vi "InitCSMs.vi"(7 "Enable Conditional Building lvlibp?":bool=TRUE, 8 "error in":errorcluster) -> (0 "error out":errorcluster, 2 "CSMs":string[](array[string]))   [LabVIEW 2017, in "CSM-Testcase.lvlib"]
uses:
  CSM-Testcase.lvlib
  <vilib>/AppBuilder/AB_API_Simple/Build (path).vi
  Chain1.vi
  Chain2.vi
  Chain3.vi
  src/user.lib/_NEVSTOP/Communicable State Machine(CSM)/Communicable State Machine.lvlib
  <vilib>/AppBuilder/AB_API_Simple/NI_App_Builder_API.lvlib
panel:
  out "Waited (ms)":u32
  out "CSMs Left":string[](array[string])
  out "Generated files":path[](array[path])
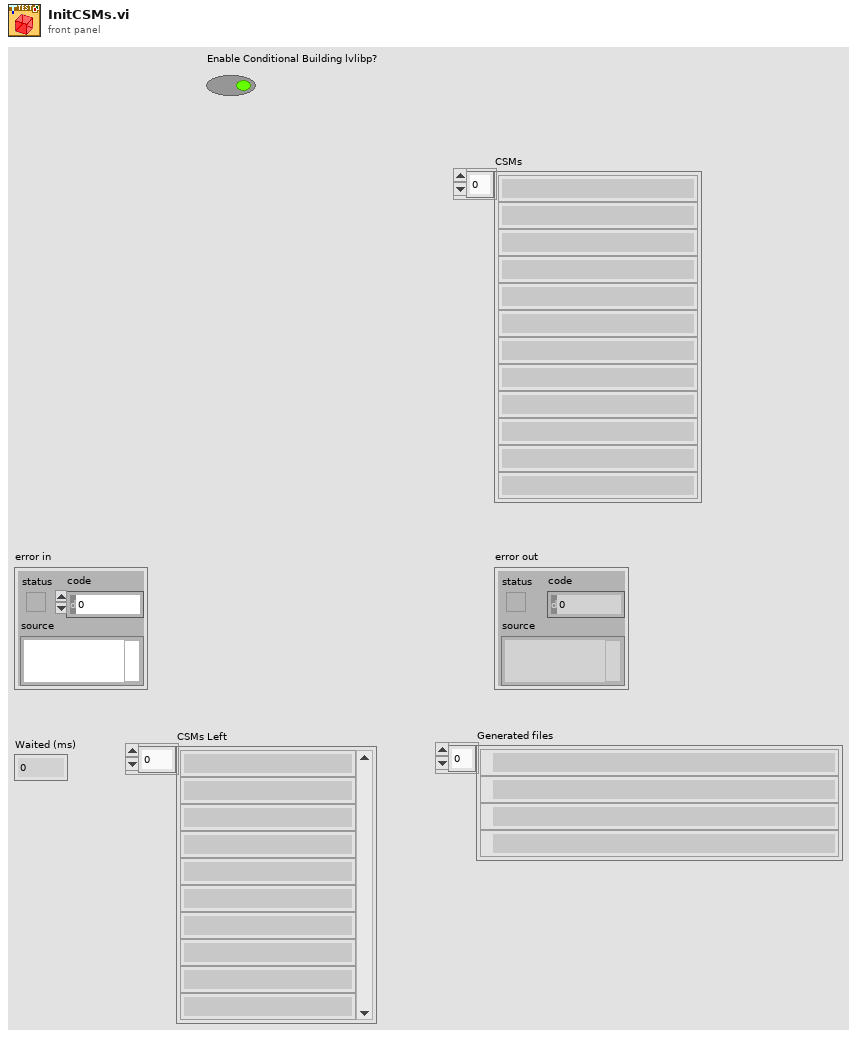
[diagram p1: front panel]
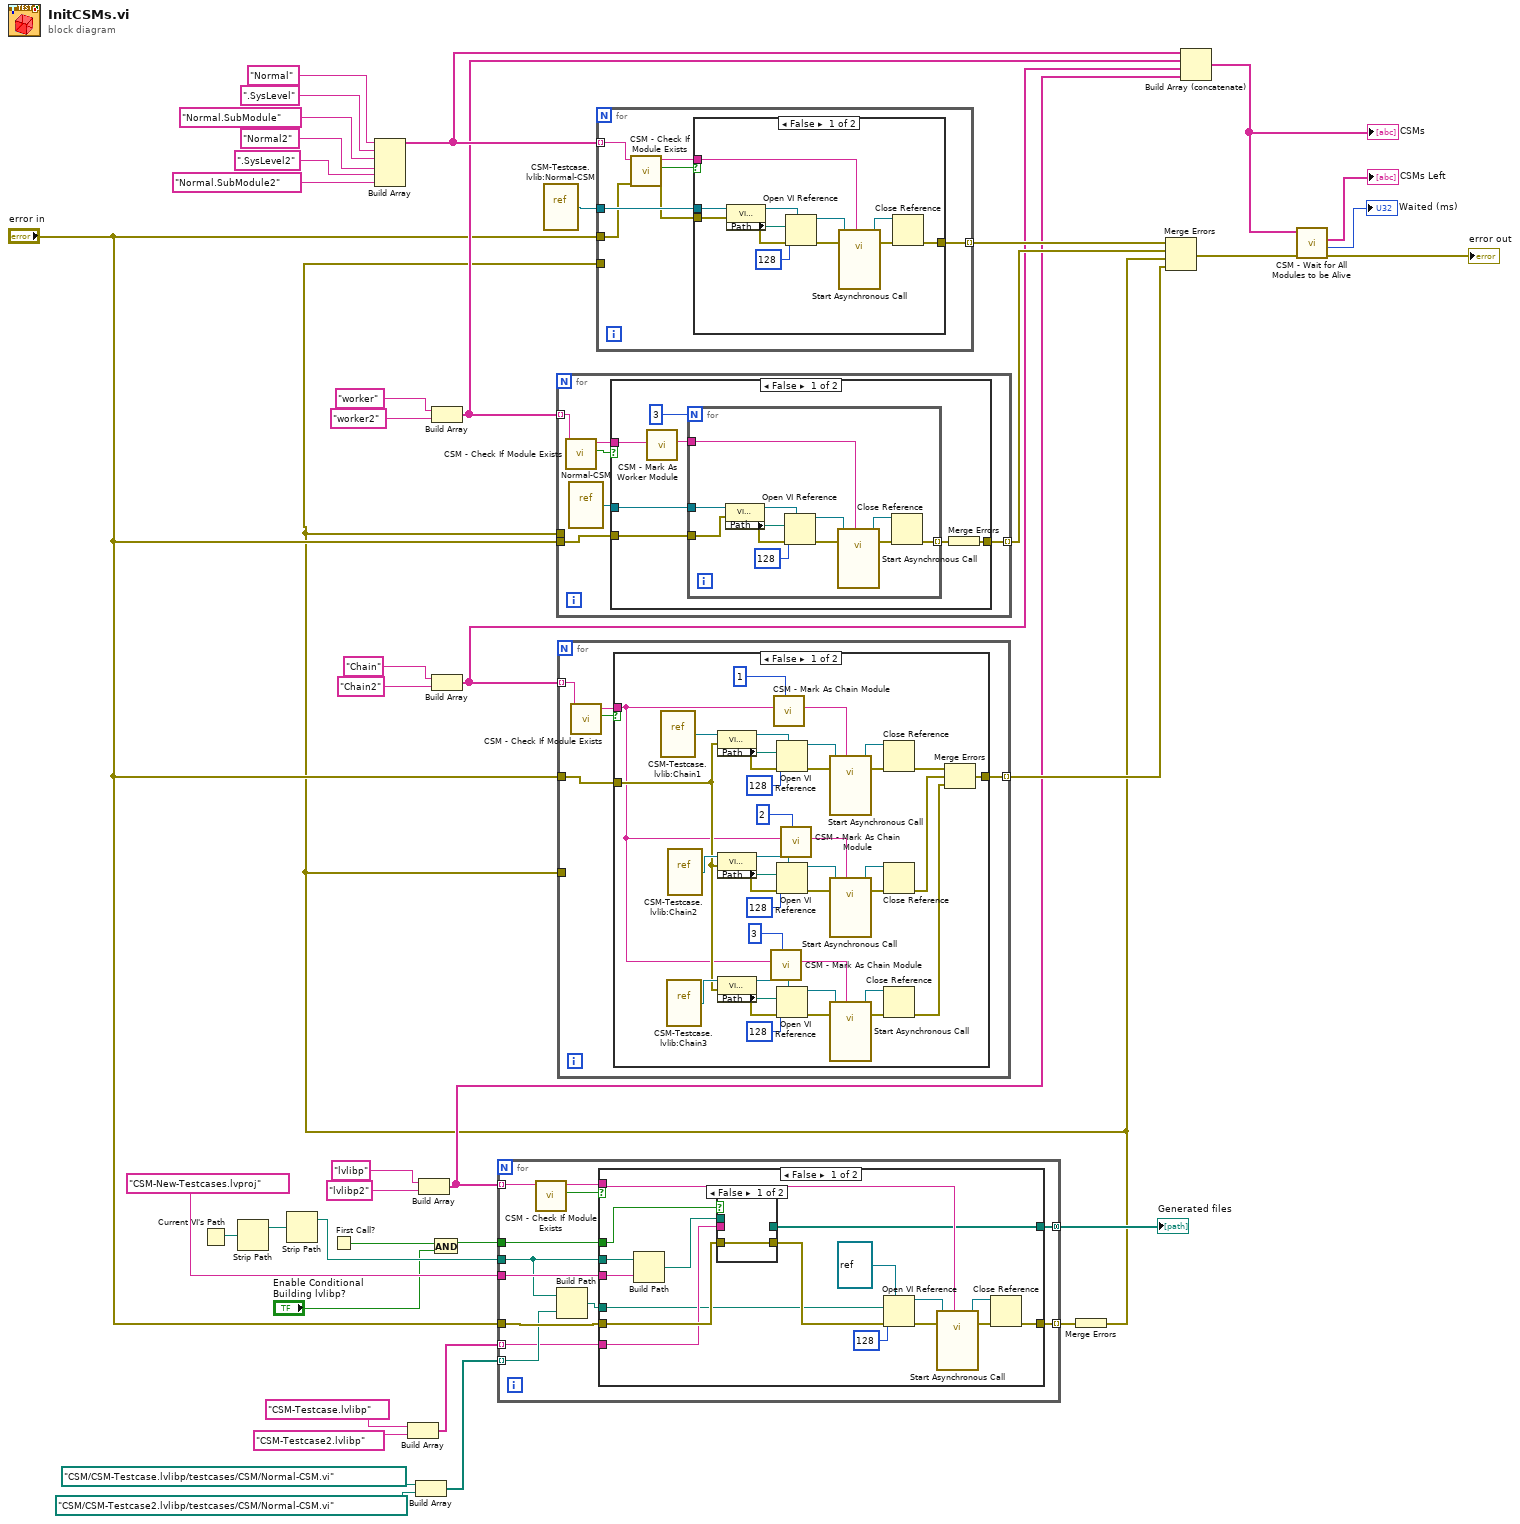
[diagram p0: block diagram]
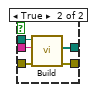
[diagram p2: hidden frame]
diagram:
  n1 = Current VI's Path() -> (path=w38:path)
  n2 = Strip Path(path=w38) -> (stripped path=w39:path)  [unwired: 1 out]
  n3 = Strip Path(path=w39) -> (stripped path=w40:path)  [unwired: 1 out]
  n4 = First Call?() -> (First Call?: T/F=w4:bool)
  n5 = Build Array("Normal" ("Name (\"\" to Use UUID)"), ".SysLevel" ("Name (\"\" to Use UUID)"), "Normal.SubModule" ("Name (\"\" to Use UUID)"), "Normal2" ("Name (\"\" to Use UUID)"), ".SysLevel2" ("Name (\"\" to Use UUID)"), "Normal.SubModule2" ("Name (\"\" to Use UUID)")) -> (w34:string[])
  n6 = Build Array("CSM-Testcase.lvlibp" ("Name of build specification (if empty: build all)"), "CSM-Testcase2.lvlibp" ("Name of build specification (if empty: build all)")) -> (w12:string[])
  n7 = Build Array(path "CSM/CSM-Testcase.lvlibp/testcases/CSM/Normal-CSM.vi" ("vi path"), path "CSM/CSM-Testcase2.lvlibp/testcases/CSM/Normal-CSM.vi" ("vi path")) -> (w15:path[])
  n8 = Build Array("lvlibp" ("Name (\"\" to Use UUID)"), "lvlibp2" ("Name (\"\" to Use UUID)")) -> (w18:string[])
  n9 = And(x=w4, y="Enable Conditional Building lvlibp?") -> (x .and. y?=w3:bool)
  n10 = Build Array("worker" ("Name (\"\" to Use UUID)"), "worker2" ("Name (\"\" to Use UUID)")) -> (w24:string[])
  n11 = Build Array("Chain" ("Name (\"\" to Use UUID)"), "Chain2" ("Name (\"\" to Use UUID)")) -> (w21:string[])
  n12 = for {
    tunnel: "CSM-New-Testcases.lvproj" ("name or relative path") -> [w52]
    tunnel: w40 -> [w47]
    tunnel: w18 -> [w49] mode=indexing
    tunnel: w15 -> [w48] mode=indexing
    tunnel: w12 -> [w45] mode=indexing
    tunnel: [w44] -> w11 mode=concatenating
    tunnel: w3 -> [w43]
    tunnel: "error in" -> [w53]
    tunnel: [w51] -> w37 mode=indexing
    n13 = call "CSM - Check If Module Exists.vi"("CSM Name"=w49) -> ("Exist?"=w54:bool, "CSM Name (Dup)"=w50:string)  [unwired: 8 in, 1 out]
    n14 = Build Path(base path=w47, name or relative path=w48) -> (appended path=w46:path)
    n15 = case shown="False" w54 {
      tunnel: [w71 w78] -> w51
      tunnel: w46 -> [w57 _]
      tunnel: w47 -> [w64 _]
      tunnel: w52 -> [w63 _]
      tunnel: w50 -> [w62 _]
      tunnel: w53 -> [w61 w78]
      tunnel: w45 -> [w59 _]
      tunnel: [w58 _] -> w44
      tunnel: w43 -> [w55 _]
      frame False {
        n16 = Build Path(base path=w64, name or relative path=w63) -> (appended path=w56:path)
        n17 = case shown="False" w55 {
          tunnel: w61 -> [w72 w77]
          tunnel: [w72 w76] -> w60
          tunnel: w59 -> [_ w75]
          tunnel: [_ w74] -> w58
          tunnel: w56 -> [_ w73]
          frame False {
          }
          frame True {
            n18 = call-poly <vilib>:"Build.vi"("error in (no error)"=w77, "Name of build specification (if empty: build all)"=w75, "Path to project"=w73) -> ("error out"=w76:errorcluster, "Generated files"=w74:path[])  [unwired: 7 in]
          }
        }
        n19 = Open VI Reference(type specifier VI Refnum (for type only)=refnum<vi> refnum ("reference out"), vi path=w57, options=128, error in (no error)=w60) -> (vi reference=w67:refnum<vi>, error out=w69:errorcluster)  [unwired: 2 in]
        n20 = call-by-ref "Start Asynchronous Call"(reference=w67, error in=w69, "Name (\"\" to Use UUID)"=w62) -> (reference out=w66:refnum<vi>, error out=w68:errorcluster)  [unwired: 11 in]
        n21 = Close Reference(reference=w66, error in (no error)=w68) -> (error out=w71:errorcluster)
      }
      frame True {
      }
    }
  }
  "Generated files" <- w11
  n22 = vi-ref "CSM-Testcase.lvlib:Normal-CSM.vi"() -> (w30:refnum<vi>)
  n23 = Merge Errors(w37) -> (w1:errorcluster)
  n24 = for {
    tunnel: w24 -> [w80] mode=indexing
    tunnel: "error in" -> [w84]
    tunnel: [w81] -> w36 mode=indexing
    tunnel: w1 -> [_]
    n25 = call "CSM - Check If Module Exists.vi"("CSM Name"=w80) -> ("Exist?"=w83:bool, "CSM Name (Dup)"=w82:string)  [unwired: 8 in, 1 out]
    n26 = vi-ref "Normal-CSM.vi"() -> (w79:refnum<vi>)
    n27 = case shown="False" w83 {
      tunnel: w79 -> [w91 _]
      tunnel: [w85 w104] -> w81
      tunnel: w84 -> [w87 w104]
      tunnel: w82 -> [w86 _]
      frame False {
        n28 = call "CSM - Mark As Worker Module.vi"("CSM Name"=w86) -> ("CSM Name (Marked As Worker)"=w88:string)  [unwired: 9 in]
        n29 = for {
          N: 3 -> [_]
          tunnel: w91 -> [w95]
          tunnel: w88 -> [w94]
          tunnel: [w93] -> w89 mode=indexing
          tunnel: w87 -> [w92]
          n30 = property class="VI (strict)"(reference=w95, error in=w92) -> (reference out=w101:refnum<vi>, error out=w99:errorcluster, "Path"=w98:path)
          n31 = Open VI Reference(type specifier VI Refnum (for type only)=w101, vi path=w98, options=128, error in (no error)=w99) -> (vi reference=w97:refnum<vi>, error out=w102:errorcluster)  [unwired: 2 in]
          n32 = call-by-ref "Start Asynchronous Call"(reference=w97, error in=w102, "Name (\"\" to Use UUID)"=w94) -> (reference out=w96:refnum<vi>, error out=w100:errorcluster)  [unwired: 11 in]
          n33 = Close Reference(reference=w96, error in (no error)=w100) -> (error out=w93:errorcluster)
        }
        n34 = Merge Errors(w89) -> (w85:errorcluster)
      }
      frame True {
      }
    }
  }
  n35 = for {
    tunnel: w21 -> [w105] mode=indexing
    tunnel: "error in" -> [w109]
    tunnel: [w107] -> w42 mode=indexing
    tunnel: w1 -> [_]
    n36 = call "CSM - Check If Module Exists.vi"("CSM Name"=w105) -> ("Exist?"=w108:bool, "CSM Name (Dup)"=w106:string)  [unwired: 8 in, 1 out]
    n37 = case shown="False" w108 {
      tunnel: [w112 w149] -> w107
      tunnel: w109 -> [w111 w149]
      tunnel: w106 -> [w110 _]
      frame False {
        n38 = vi-ref "CSM-Testcase.lvlib:Chain1.vi"() -> (w148:refnum<vi>)
        n39 = vi-ref "CSM-Testcase.lvlib:Chain3.vi"() -> (w130:refnum<vi>)
        n40 = vi-ref "CSM-Testcase.lvlib:Chain2.vi"() -> (w131:refnum<vi>)
        n41 = property class="VI (strict)"(reference=w148, error in=w111) -> (reference out=w145:refnum<vi>, error out=w143:errorcluster, "Path"=w142:path)
        n42 = property class="VI (strict)"(reference=w131, error in=w111) -> (reference out=w134:refnum<vi>, error out=w136:errorcluster, "Path"=w137:path)
        n43 = property class="VI (strict)"(reference=w130, error in=w111) -> (reference out=w127:refnum<vi>, error out=w125:errorcluster, "Path"=w124:path)
        n44 = call "CSM - Mark As Chain Module.vi"("Order"=3, "CSM Name"=w110) -> ("CSM Name (Marked As Chain)"=w118:string)  [unwired: 8 in]
        n45 = call "CSM - Mark As Chain Module.vi"("Order"=1, "CSM Name"=w110) -> ("CSM Name (Marked As Chain)"=w116:string)  [unwired: 8 in]
        n46 = Open VI Reference(type specifier VI Refnum (for type only)=w145, vi path=w142, options=128, error in (no error)=w143) -> (vi reference=w141:refnum<vi>, error out=w146:errorcluster)  [unwired: 2 in]
        n47 = Open VI Reference(type specifier VI Refnum (for type only)=w134, vi path=w137, options=128, error in (no error)=w136) -> (vi reference=w138:refnum<vi>, error out=w133:errorcluster)  [unwired: 2 in]
        n48 = Open VI Reference(type specifier VI Refnum (for type only)=w127, vi path=w124, options=128, error in (no error)=w125) -> (vi reference=w123:refnum<vi>, error out=w128:errorcluster)  [unwired: 2 in]
        n49 = call "CSM - Mark As Chain Module.vi"("Order"=2, "CSM Name"=w110) -> ("CSM Name (Marked As Chain)"=w117:string)  [unwired: 8 in]
        n50 = call-by-ref "Start Asynchronous Call"(reference=w141, error in=w146, "Name (\"\" to Use UUID)"=w116) -> (reference out=w140:refnum<vi>, error out=w144:errorcluster)  [unwired: 11 in]
        n51 = call-by-ref "Start Asynchronous Call"(reference=w138, error in=w133, "Name (\"\" to Use UUID)"=w117) -> (reference out=w139:refnum<vi>, error out=w135:errorcluster)  [unwired: 11 in]
        n52 = call-by-ref "Start Asynchronous Call"(reference=w123, error in=w128, "Name (\"\" to Use UUID)"=w118) -> (reference out=w122:refnum<vi>, error out=w126:errorcluster)  [unwired: 11 in]
        n53 = Close Reference(reference=w140, error in (no error)=w144) -> (error out=w121:errorcluster)
        n54 = Close Reference(reference=w139, error in (no error)=w135) -> (error out=w120:errorcluster)
        n55 = Close Reference(reference=w122, error in (no error)=w126) -> (error out=w119:errorcluster)
        n56 = Merge Errors(w121, w120, w119) -> (w112:errorcluster)
      }
      frame True {
      }
    }
  }
  n57 = for {
    tunnel: w30 -> [w156]
    tunnel: w34 -> [w152] mode=indexing
    tunnel: [w155] -> w35 mode=indexing
    tunnel: "error in" -> [w154]
    tunnel: w1 -> [_]
    n58 = call "CSM - Check If Module Exists.vi"("Error In"=w154, "CSM Name"=w152) -> ("error out"=w153:errorcluster, "Exist?"=w150:bool, "CSM Name (Dup)"=w151:string)  [unwired: 7 in]
    n59 = case shown="False" w150 {
      tunnel: w156 -> [w160 _]
      tunnel: [w159 w169] -> w155
      tunnel: w153 -> [w158 w169]
      tunnel: w151 -> [w157 _]
      frame False {
        n60 = property class="VI (strict)"(reference=w160, error in=w158) -> (reference out=w166:refnum<vi>, error out=w164:errorcluster, "Path"=w163:path)
        n61 = Open VI Reference(type specifier VI Refnum (for type only)=w166, vi path=w163, options=128, error in (no error)=w164) -> (vi reference=w162:refnum<vi>, error out=w167:errorcluster)  [unwired: 2 in]
        n62 = call-by-ref "Start Asynchronous Call"(reference=w162, error in=w167, "Name (\"\" to Use UUID)"=w157) -> (reference out=w161:refnum<vi>, error out=w165:errorcluster)  [unwired: 11 in]
        n63 = Close Reference(reference=w161, error in (no error)=w165) -> (error out=w159:errorcluster)
      }
      frame True {
      }
    }
  }
  n64 = Merge Errors(w35, w36, w1, w42) -> (w10:errorcluster)
  n65 = Build Array (concatenate)(w34, w24, w21, w18) -> (w9:string[])
  "CSMs" <- w9
  n66 = call "CSM - Wait for All Modules to be Alive.vi"("Error In"=w10, "CSM Names"=w9) -> ("error out"=→"error out":errorcluster, "Waited (ms)"=→"Waited (ms)":u32, "CSMs Left"=→"CSMs Left":string[])  [unwired: 7 in]
